vi "Climb Controller.vi"(8 "error in":errorcluster) -> ()   [LabVIEW 2025]
doc: "This VI executes continuously carrying out the current operation and responding to updates or new operations. It will often contain the timing or control code that is difficult to place directly in TeleOp. This VI generally opens all sensors and motors and isolates the rest of the robot code from knowing how the operations are carried out."
uses:
  <vilib>/Rock Robotics/WPI/ThirdParty/REV Robotics/REVLib/Typedef/SPARK PID Gains.ctl
  <vilib>/Rock Robotics/WPI/ThirdParty/REV Robotics/REVLib/Typedef/SPARK Feed Forward Gains.ctl
  Climb Setpoints.ctl
  Climb Operations.ctl
  <vilib>/Rock Robotics/WPI/ThirdParty/REV Robotics/REVLib/Typedef/Spark MAX Control Type.ctl
  724bb587-651a-46f3-9bc9-aa29472fbfc3.vi
  a54b9f28-b9ad-4612-aeb9-ad182f8790f4.vi
  <vilib>/Rock Robotics/WPI/ThirdParty/REV Robotics/REVLib/SubVI/Public/SPARK Open Brushless.vi
  <vilib>/Rock Robotics/WPI/ThirdParty/REV Robotics/REVLib/SubVI/Public/SPARK Get Encoder Status Position.vi
  <vilib>/Rock Robotics/WPI/ThirdParty/REV Robotics/REVLib/SubVI/Public/SPARK Configure Closed Loop Gains.vi
  <vilib>/Rock Robotics/WPI/ThirdParty/REV Robotics/REVLib/SubVI/Public/SPARK Configure Closed Loop Output Range.vi
  <vilib>/Rock Robotics/Network Tables/NT Write Boolean.vi
panel:
  out "Climb":cluster{"Climb Pos":dbl, "Sensor Velocity":dbl}(graph)
  in  "Climb Pos":dbl=-200.0
  in  "Min Out Climb":dbl=-1.0
  in  "Max Out Climb":dbl=1.0
  in  "FF Gains Climb":T1
  in  "PID Gains Climb":T2={"kP"=0.03, "kI"=0.0, "kD"=0.0}
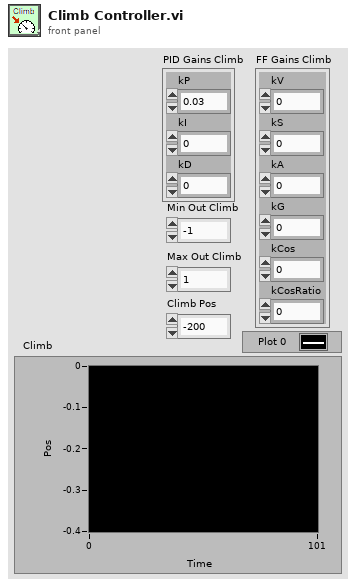
[diagram p1: front panel]
types:
  T1 = typedef "SPARK Feed Forward Gains.ctl" = cluster{"kV":dbl, "kS":dbl, "kA":dbl, "kG":dbl, "kCos":dbl, "kCosRatio":dbl}
  T2 = typedef "SPARK PID Gains.ctl" = cluster{"kP":dbl, "kI":dbl, "kD":dbl}
  T3 = typedef "Climb Setpoints.ctl" = cluster{"Operation":T4, "Climb":bool}
  T4 = typedef "Climb Operations.ctl" = enum16{"Reserve", "Read Current", "Immediate", "Control the climb hook, and the hopper extension"}
  T5 = typedef "WPI_MotorControlDeviceRef.ctl" = cluster{"DeviceStatus":errorcluster, "Type":T6, "PWM":cluster{"PWM Channel":T7, "DeadBand":T8}, "CAN":cluster{"Device Number":u8, "SetOutput VI Ref":variant, "GetOutput VI Ref":variant, "Enable VI Ref":variant, "Disable VI Ref":variant, "Data":variant}, "Invert":bool, "DIO PWM":cluster{"PWM \"Enable\" Channel":T7, "DIOChannel":T9, "PWM Rate":dbl}}
  T6 = typedef "WPI_MotorControlType.ctl" = enum16{"PWM", "CAN", "DIO PWM"}
  T7 = typedef "FPGA_DIOPWMChannel.ctl" = enum8{"PWM 0", "PWM 1", "PWM 2", "PWM 3", "PWM 4", "PWM 5", "PWM 6", "PWM 7", "PWM 8", "PWM 9", "PWM MXP 0", "PWM MXP 1", "PWM MXP 2", "PWM MXP 3", "PWM MXP 4", "PWM MXP 5", "PWM MXP 6", "PWM MXP 7", "PWM MXP 8", "PWM MXP 9", "Invalid"}
  T8 = typedef "WPI_PWMDeadband.ctl" = cluster{"Name":string, "maxPositivePwm":i32, "minPositivePwm":i32, "centerPwm":i32, "maxNegativePwm":i32, "minNegativePwm":i32, "angularRange":u16}
  T9 = typedef "FPGA_DIOChannel.ctl" = enum8{"DIO 0", "DIO 1", "DIO 2", "DIO 3", "DIO 4", "DIO 5", "DIO 6", "DIO 7", "DIO 8", "DIO 9", "DIO MXP 0", "DIO MXP 1", "DIO MXP 2", "DIO MXP 3", "DIO MXP 4", "DIO MXP 5", "DIO MXP 6", "DIO MXP 7", "DIO MXP 8", "DIO MXP 9", "DIO MXP 10", "DIO MXP 11", "DIO MXP 12", "DIO MXP 13", "DIO MXP 14", "DIO MXP 15", "SPI Port CS1", "SPI Port CS2", "SPI Port CS3", "SPI Port MISO", "SPI Port MOSI", "Invalid"}
  T10 = typedef "Command Status Info.ctl" = cluster{"Name":string, "Status":T11, "notifier out":T12}
  T11 = typedef "Completion Status.ctl" = enum16{"Successful", "Aborted", "Incomplete"}
  T12 = typedef "Completion Notifier.ctl" = refnum<notifier>
  T13 = cluster{"Current Command":T3, "Command Timing":cluster{"Start Time (ms)":u32, "Iterations":i32}, "Command Arguments":cluster{"Command Info":T10, "Description":string, "Default Command":T3, "queue out":refnum<queue>, "Subsystem Name":string}}
  T14 = typedef "Spark MAX Control Type.ctl" = enum16{"Percent VBus", "Voltage", "Velocity", "Position", "Smart Motion", "Current", "Smart Velocity", "MAXMotion Position", "MAXMotion Velocity"}
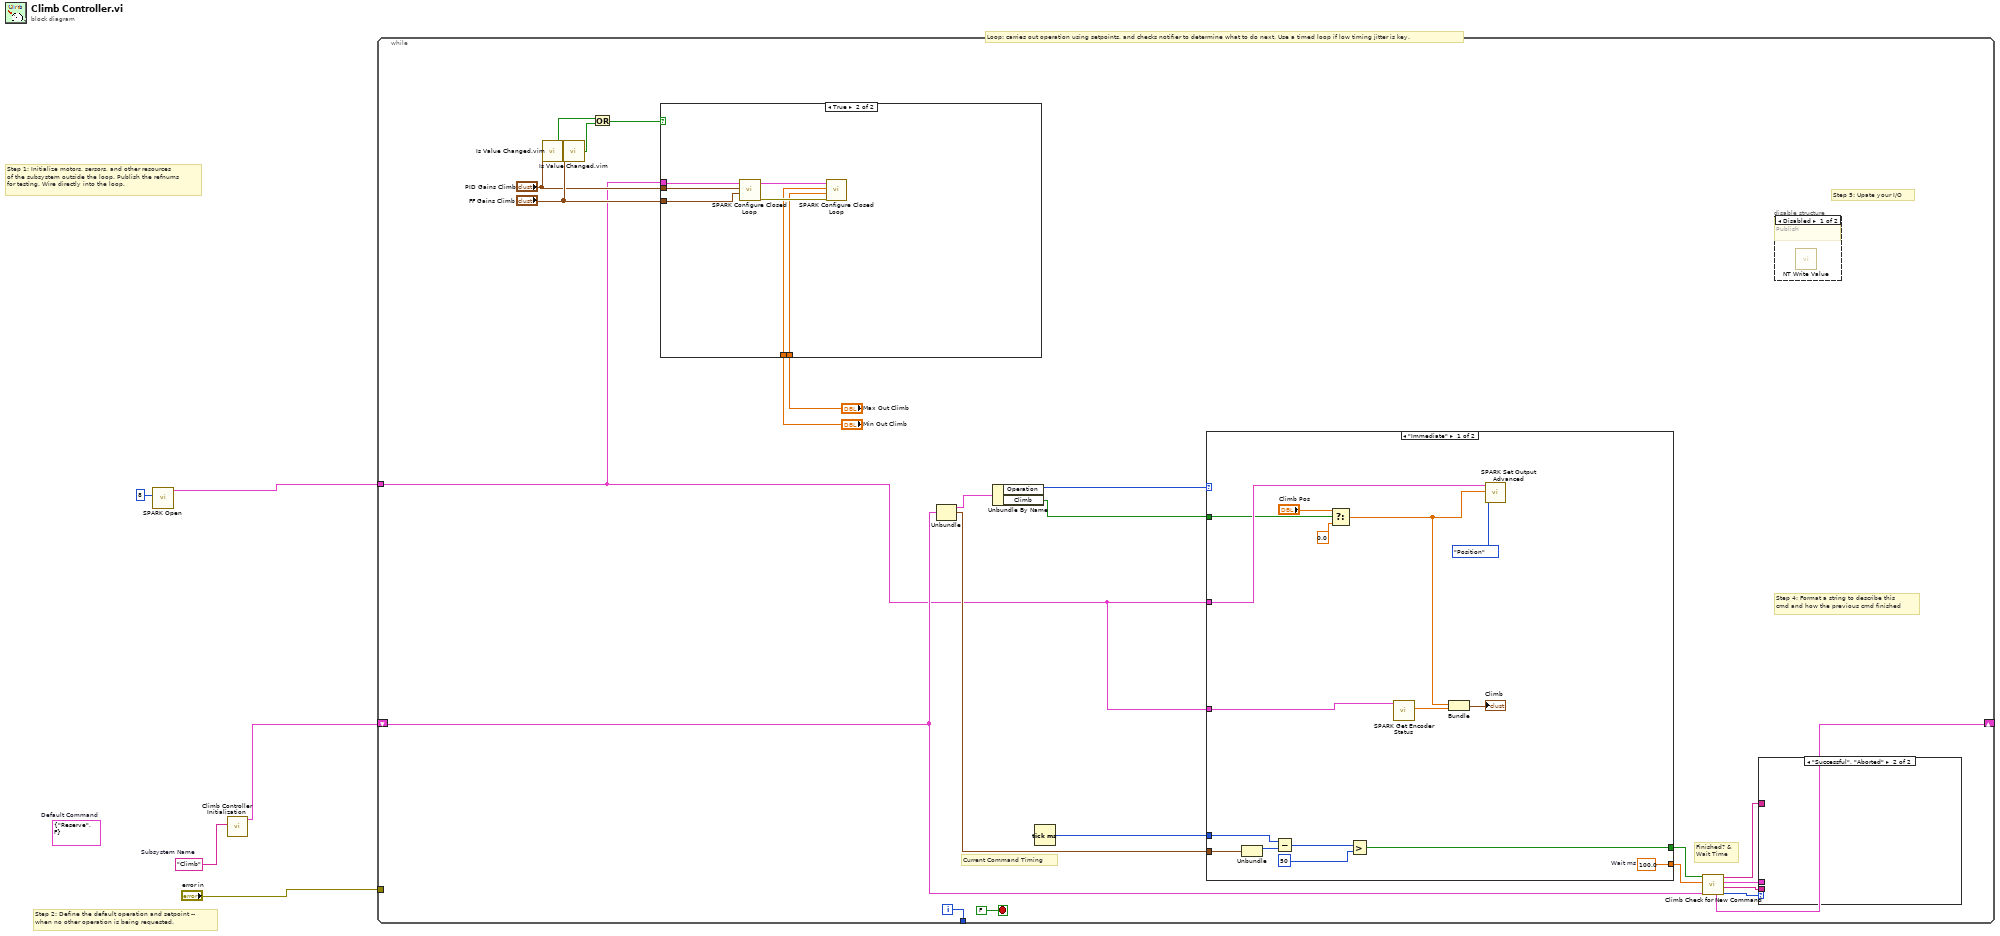
[diagram p0: block diagram]
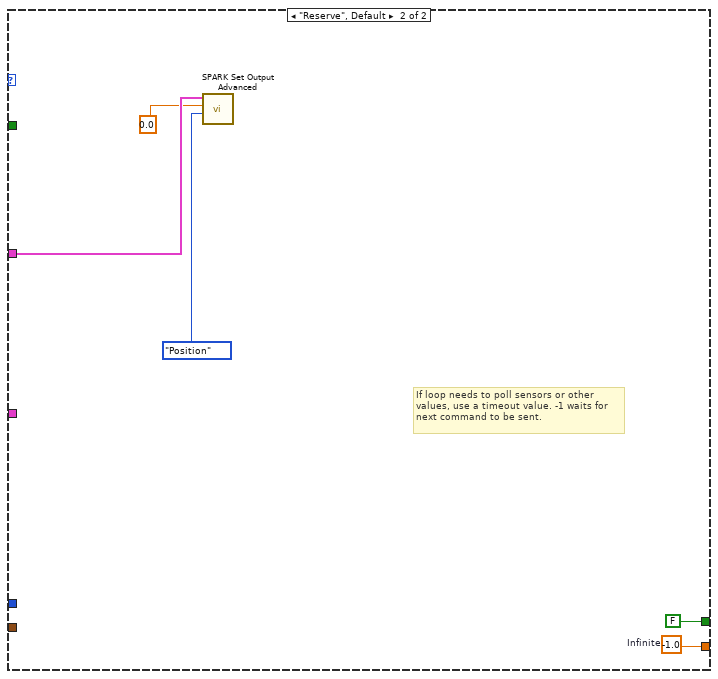
[diagram p5: hidden frame]
diagram:
  (unwired) T3 {"Operation"=enum."Reserve", "Climb"=FALSE}  # Default Command
  w3 = "Climb"  # Subsystem Name
  # "Step 2: Define the default operation and setpoint --\nwhen no other operation is being requested."
  # "Step 1: Initialize motors, sersors, and other resources\nof the subsystem outside the loop. Publish the refnums\nfor testing. Wire directly into the loop."
  # "Loop: carries out operation using setpoints, and checks notifier to determine what to do next. Use a timed loop if low timing jitter is key."
  n1 = call-poly <vilib>:"SPARK Open.vi"("Device Number"=u8 8) -> ("MotorControlDeviceRef"=w1:T5)  [unwired: 9 in, 1 out]
  n2 = call "Climb Controller Initialization.vi"("Subsystem Name"=w3) -> ("Current Command"=w4:T13)  [unwired: 10 in]
  n3 = while {
    shift-right: [w22] -> _
    shift-left: w4 -> [w15]
    tunnel: [w27] -> _
    tunnel: "error in" -> [_]
    tunnel: w1 -> [w8]
    i -> [w27]
    stop <- FALSE stop-if-true
    # "Step 5: Upate your I/O"
    # "Step 4: Format a string to describe this\ncmd and how the previous cmd finished"
    # "Current Command Timing"
    # "Finished? &\nWait Time"
    n4 = call "Is Value Changed.vim"("value"="PID Gains Climb") -> ("changed or first call?"=w6:bool)
    n5 = call "Is Value Changed.vim"("value"="FF Gains Climb") -> ("changed or first call?"=w7:bool)
    n6 = Or(x=w6, y=w7) -> (x .or. y?=w14:bool)
    n7 = case shown="True" w14 {
      tunnel: w8 -> [_ w33]
      tunnel: "PID Gains Climb" -> [_ w32]
      tunnel: "FF Gains Climb" -> [_ w31]
      tunnel: "Max Out Climb" -> [_ w30]
      tunnel: "Min Out Climb" -> [_ w29]
      frame False {
      }
      frame True {
        n8 = call-poly <vilib>:"SPARK Configure Closed Loop.vi"("Feed Forward Gains"=w31, "PID Gains"=w32, "MotorControlDeviceRef in"=w33) -> ("error out"=w35:errorcluster, "MotorControlDeviceRef out"=w34:T5)  [unwired: 7 in]
        n9 = call-poly <vilib>:"SPARK Configure Closed Loop.vi"("error in"=w35, "Maximum Output"=w30, "Minimum Output"=w29, "MotorControlDeviceRef in"=w34) -> ()  [unwired: 6 in, 2 out]
      }
    }
    n10 = Unbundle(w15) -> ("Current Command"=w26:T3, "Command Timing"=w23:cluster{"Start Time (ms)":u32, "Iterations":i32})  [unwired: 1 out]
    n11 = Unbundle By Name(w26) -> ("Operation"=w25:T4, "Climb"=w9:bool)
    n12 = Tick Count (ms)() -> (millisecond timer value=w24:u32)
    n13 = case shown="\"Immediate\"" w25 {
      tunnel: [w51 w56] -> w20
      tunnel: [w45 FALSE ("ignore previous (F)")] -> w21
      tunnel: w23 -> [w47 _]
      tunnel: w24 -> [w46 _]
      tunnel: w8 -> [w44 w54]
      tunnel: w9 -> [w41 _]
      tunnel: w8 -> [w38 _]
      frame "Immediate" {
        w51 = 100.0  # Wait ms
        n14 = Unbundle(w47) -> ("Start Time (ms)"=w50:u32)  [unwired: 1 out]
        n15 = Subtract(x=w46, y=w50) -> (x-y=w49:u32)
        n16 = Select(t="Climb Pos", s=w41, f=0.0) -> (s? t:f=w37:dbl)
        n17 = Greater?(x=w49, y=u8 50 ("Left Motor")) -> (0:w45:bool)
        n18 = call-poly <vilib>:"SPARK Get Encoder Status.vi"("MotorControlDevRef in"=w38) -> ("Sensor Position"=w40:dbl)  [unwired: 7 in, 3 out]
        n19 = Bundle("f"=w37, "Sensor Position"=w40) -> (→"Climb":cluster{"f":dbl, "Sensor Position":dbl})  [unwired: 1 in]
        n20 = call <vilib>:"SPARK Set Output Advanced.vi"("Control Mode"=Spark_MAX_Control_Type."Position", "Setpoint"=w37, "MotorControlDevRef"=w44) -> ()  [unwired: 7 in, 2 out]
      }
      frame "Reserve", Default {
        w56 = -1.0  # Infinite
        # "If loop needs to poll sensors or other\nvalues, use a timeout value. -1 waits for\nnext command to be sent."
        n21 = call <vilib>:"SPARK Set Output Advanced.vi"("Control Mode"=Spark_MAX_Control_Type."Position", "Setpoint"=0.0, "MotorControlDevRef"=w54) -> ()  [unwired: 7 in, 2 out]
      }
    }
    n22 = call "Climb Check for New Command.vi"("Current Command"=w15, "Wait time (ms)"=w20, "Finished?"=w21) -> ("Completion"=w16:T11, "Subsystem Name"=w17:string, "Current Command"=w18:T3, "Initial Trace String"=w19:string, "NextCommand"=w22:T13)  [unwired: 4 in]
    n23 = case shown="\"Successful\", \"Aborted\"" w16 {
      tunnel: w19 -> [_ _]
      tunnel: w18 -> [_ _]
      tunnel: w17 -> [_ _]
      frame "Incomplete", Default {
        # "Continuing current command"
      }
      frame "Successful", "Aborted" {
        # "Report and setup for next command"
      }
    }
    n24 = disable-structure shown="Disabled" {
      frame Disabled {
        # "Publish"
        n25 = call-poly <vilib>:"NT Write Value.vi"() -> ()  [unwired: 11 in, 1 out]
      }
      frame Enabled {
      }
    }
  }
